vi "Fetch.vi"(8 "错误输入":errorcluster caption="错误输入（无错误）", 10 "Command":string="hello", 11 "VISA资源":refnum<visa-resource-name>) -> (0 "错误输出":errorcluster, 1 "数值":dbl, 2 "成功？":bool, 3 "VISA资源":refnum<visa-resource-name>, 4 "结果字符串":string, 5 "返回指令":string)   [LabVIEW 2026, in "UI-Zolix.lvlib"]
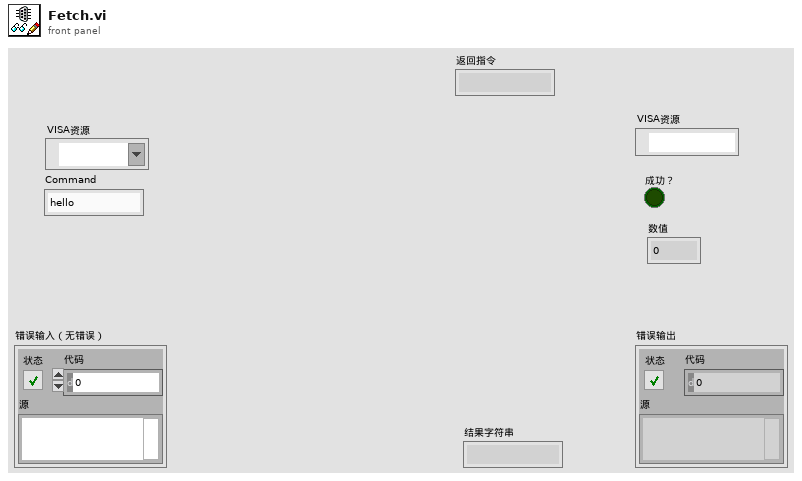
[diagram p1: front panel]
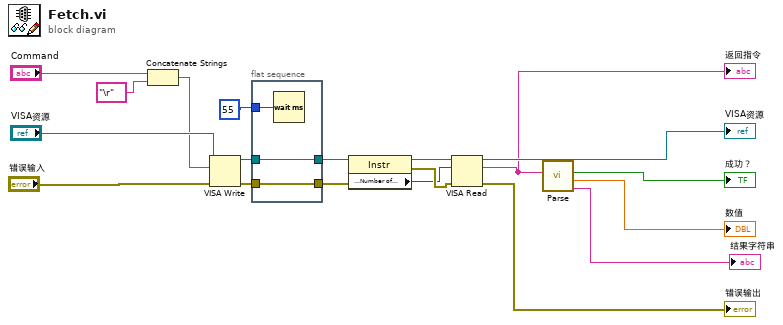
[diagram p0: block diagram]
diagram:
  n1 = Concatenate Strings("Command", "\r" ("字符串")) -> (w6:string)
  n2 = VISA Write(VISA resource name="VISA资源", write buffer=w6, error in (no error)="错误输入") -> (VISA resource name out=w17:refnum<visa-resource-name>, error out=w19:errorcluster)  [unwired: 1 out]
  n3 = flat-sequence {
    tunnel: w19 -> [w21]
    tunnel: [w21] -> w18
    tunnel: w17 -> [w20]
    tunnel: [w20] -> w16
    tunnel: u32 55 ("读取前延时(ms)") -> [w22]
    frame #0 {
      n4 = Wait (ms)(milliseconds to wait=w22) -> ()  [unwired: 1 out]
    }
  }
  n5 = property class="Instr"(reference=w16, error in=w18) -> (reference out=w13:refnum<visa-resource-name>, error out=w12:errorcluster, "Serial Settings:Number of Bytes at Serial Port"=w11:u32)
  n6 = VISA Read(VISA resource name=w13, byte count=w11, error in (no error)=w12) -> (VISA resource name out=→"VISA资源":refnum<visa-resource-name>, read buffer=w2:string, error out=→"错误输出":errorcluster)  [unwired: 1 out]
  "返回指令" <- w2
  n7 = call "Parse.vi"("命令"=w2) -> ("结果字符串"=→"结果字符串":string, "数字"=→"数值":dbl, "成功？"=→"成功？":bool)  [unwired: 8 in]
